vi "Cleanup.vi"(8 "error in (no error)":errorcluster, 11 "SequenceViewPanel in":refnum<class "SequenceViewPanel.lvclass">) -> (0 "error out":errorcluster)   [LabVIEW 2020, in "TSnax UI.lvlib" / "SequenceViewPanel.lvclass"]
uses:
  SequenceViewPanel.lvclass
  SequenceViewPanel.lvclass/SequenceViewPanel.ctl
  <vilib>/IlluminatedG/IG OOPanel/OOPanel/Panel/Panel.lvclass
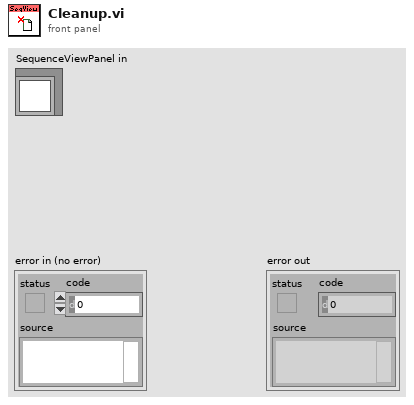
[diagram p1: front panel]
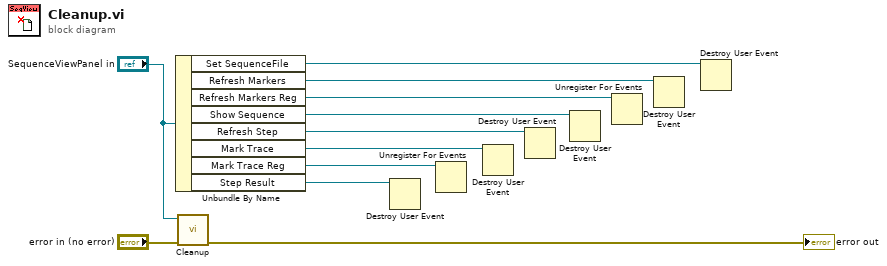
[diagram p0: block diagram]
diagram:
  n1 = Unbundle By Name("SequenceViewPanel in") -> ("Set SequenceFile"=w11:refnum<user-event>, "Refresh Markers"=w6:refnum<user-event>, "Refresh Markers Reg"=w7:refnum<event-registration>, "Show Sequence"=w5:refnum<user-event>, "Refresh Step"=w4:refnum<user-event>, "Mark Trace"=w3:refnum<user-event>, "Mark Trace Reg"=w2:refnum<event-registration>, "Step Result"=w1:refnum<user-event>)
  n2 = call-parent "Cleanup.vi"("error in (no error)"="error in (no error)", "Panel in"="SequenceViewPanel in") -> ("error out"=→"error out":errorcluster)  [unwired: 9 in]
  n3 = Destroy User Event(user event=w1) -> ()  [unwired: 1 in, 1 out]
  n4 = Unregister For Events(event registration refnum=w2) -> ()  [unwired: 1 in, 1 out]
  n5 = Destroy User Event(user event=w3) -> ()  [unwired: 1 in, 1 out]
  n6 = Destroy User Event(user event=w4) -> ()  [unwired: 1 in, 1 out]
  n7 = Destroy User Event(user event=w5) -> ()  [unwired: 1 in, 1 out]
  n8 = Unregister For Events(event registration refnum=w7) -> ()  [unwired: 1 in, 1 out]
  n9 = Destroy User Event(user event=w6) -> ()  [unwired: 1 in, 1 out]
  n10 = Destroy User Event(user event=w11) -> ()  [unwired: 1 in, 1 out]
